vi "Configure Session.vi"(8 "error in":errorcluster, 11 "Plugin in":refnum<class "NVH Condition Indicators.lvclass">) -> (0 "error out":errorcluster, 3 "Plugin out":refnum<class "NVH Condition Indicators.lvclass">)   [LabVIEW 2026, in "NVH Condition Indicators.lvlib" / "NVH Condition Indicators.lvclass"]
uses:
  NVH Condition Indicators.lvclass
  C:/Program Files/National Instruments/LabVIEW 2026/vi.lib/FlexLogger/SDK/PluginSDK.lvlibp/PEFClasses/SDK/Plugin/Plugin.lvclass
  NVH Condition Indicators.lvclass/NVH Condition Indicators.ctl
  <vilib>/FlexLogger/SDK/PluginSDK.lvlibp/PEFClasses/SDK/Plugin/ParameterAccess/Read String.vi
  C:/Program Files/National Instruments/LabVIEW 2026/vi.lib/FlexLogger/SDK/PluginSDK.lvlibp/PEFClasses/SDK/Processing Element/Processing Element.lvclass
  <vilib>/FlexLogger/SDK/PluginSDK.lvlibp/PEFClasses/SDK/Plugin/Plugin.lvclass
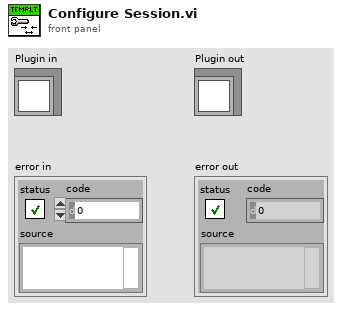
[diagram p1: front panel]
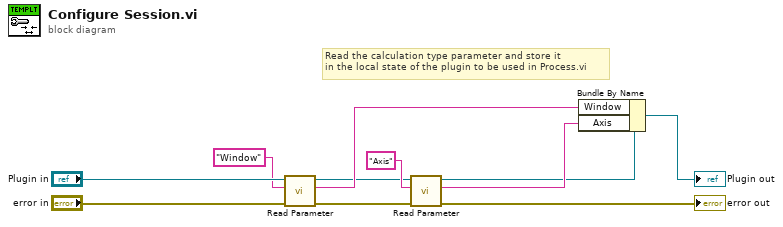
[diagram p0: block diagram]
diagram:
  # "Read the calculation type parameter and store it\nin the local state of the plugin to be used in Process.vi"
  n1 = call-poly <vilib>:"Read Parameter.vi"("error in (no error)"="error in", "Name"="Window", "Plugin in"="Plugin in") -> ("error out"=w6:errorcluster, "Value"=w7:string, "Plugin out"=w3:refnum<class "NVH Condition Indicators.lvclass">)  [unwired: 5 in, 1 out]
  n2 = call-poly <vilib>:"Read Parameter.vi"("error in (no error)"=w6, "Name"="Axis", "Plugin in"=w3) -> ("error out"=→"error out":errorcluster, "Value"=w4:string, "Plugin out"=w2:refnum<class "NVH Condition Indicators.lvclass">)  [unwired: 5 in, 1 out]
  n3 = Bundle By Name(cluster=w2, "Window"=w7, "Axis"=w4) -> (→"Plugin out":refnum<class "NVH Condition Indicators.lvclass">)
